vi "Test Properties Report.vi"() -> ()   [LabVIEW 2020]
uses:
  classes/Test Result/Node Results (Extended).ctl
  classes/Test Result/Test Node (Extended).ctl
  classes/Test Result/Test Registration Data.ctl
  classes/Test Result/Assert Event Data (Extended).ctl
  classes/Test Suite/Define Test Suite (JUnit Report).vi
  classes/Test Suite/Define Test Suite (SimpleText Report).vi
  classes/Test Suite/Test Suite.lvclass
  classes/Test Result/Test Result.lvclass
panel:
  out "% Requirement Coverage":dbl
  out "report path":path
  in  "Report Format":enum16{"Basic Text Report", "JUnit Report"}(ring)
  out "Test Results":T1[](array[typedef])
  in  "error in (no error)":errorcluster
  out "error out":errorcluster
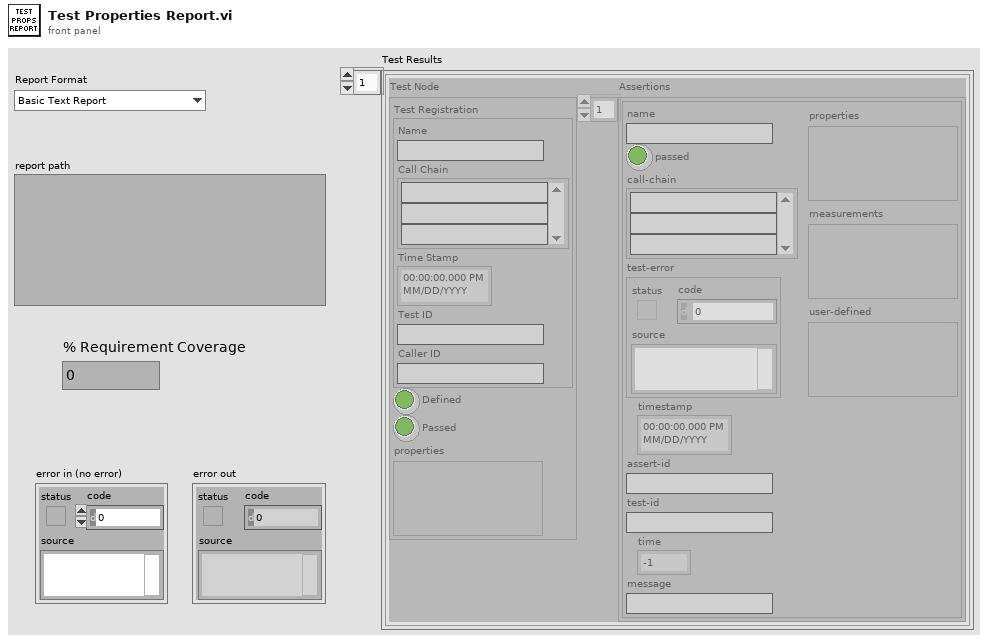
[diagram p1: front panel]
types:
  T1 = typedef "Caraya.lvlib/Test Result.lvclass/Node Results (Extended).ctl" = cluster{"Test Node":T2, "Assertions":T4[]}
  T2 = typedef "Caraya.lvlib/Test Result.lvclass/Test Node (Extended).ctl" = cluster{"Test Registration":T3, "Defined":bool, "Passed":bool, "properties":variant}
  T3 = typedef "Caraya.lvlib/Test Result.lvclass/Test Registration Data.ctl" = cluster{"Name":string, "Call Chain":string[], "Time Stamp":timestamp, "Test ID":string, "Caller ID":string}
  T4 = typedef "Caraya.lvlib/Test Result.lvclass/Assert Event Data (Extended).ctl" = cluster{"name":string, "passed":bool, "call-chain":string[], "test-error":errorcluster, "timestamp":timestamp, "assert-id":string, "test-id":string, "time":dbl, "message":string, "properties":variant, "measurements":variant, "user-defined":variant}
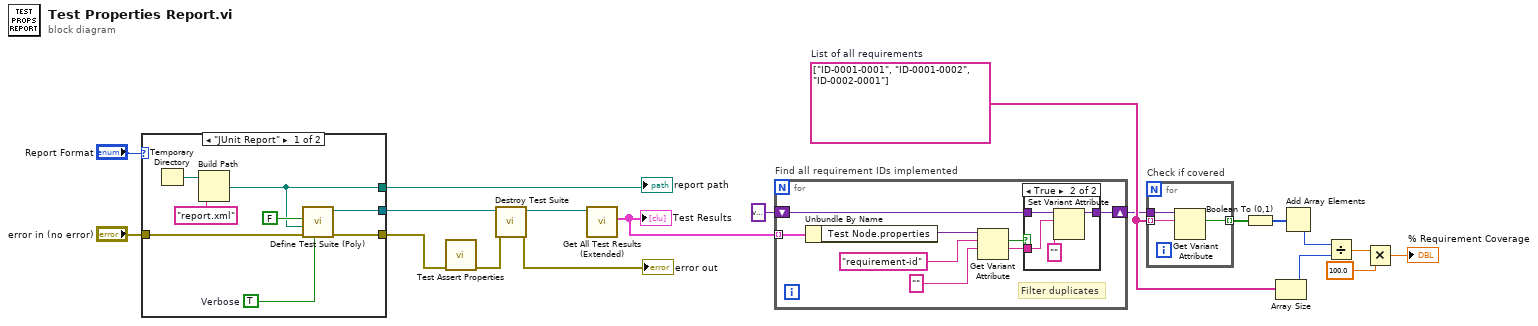
[diagram p0: block diagram]
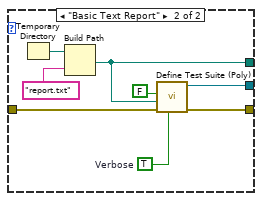
[diagram p3: hidden frame]
diagram:
  w7 = string[] ["ID-0001-0001", "ID-0001-0002", "ID-0002-0001"]  # List of all requirements
  n1 = case shown="\"JUnit Report\"" "Report Format" {
    tunnel: [w25 w35] -> w15
    tunnel: [w22 w32] -> w14
    tunnel: "error in (no error)" -> [w21 w29]
    tunnel: [w20 w28] -> w12
    frame "JUnit Report" {
      w23 = TRUE  # Verbose
      n2 = Temporary Directory() -> (w27:path)
      n3 = Build Path(base path=w27, name or relative path="report.xml") -> (appended path=w22:path)
      n4 = call-poly "Define Test Suite (Poly).vi"("Verbose (F)"=w23, "error in (no error)"=w21, "Report Path"=w22, "Interactive"=FALSE) -> ("error out"=w20:errorcluster, "Test Suite"=w25:refnum<class "Test Suite.lvclass">)  [unwired: 5 in, 1 out]
    }
    frame "Basic Text Report" {
      w31 = TRUE  # Verbose
      n5 = Temporary Directory() -> (w34:path)
      n6 = Build Path(base path=w34, name or relative path="report.txt") -> (appended path=w32:path)
      n7 = call-poly "Define Test Suite (Poly).vi"("Verbose (F)"=w31, "error in (no error)"=w29, "Report Path"=w32, "Interactive"=FALSE) -> ("error out"=w28:errorcluster, "Test Suite"=w35:refnum<class "Test Suite.lvclass">)  [unwired: 5 in, 1 out]
    }
  }
  "report path" <- w14
  n8 = call "Test Assert Properties.vi"("error in (no error)"=w12) -> ("error out"=w17:errorcluster)  [unwired: 10 in]
  n9 = call-dynamic "Destroy Test Suite.vi"("error in (no error)"=w17, "Test Suite in"=w15) -> ("error out"=→"error out":errorcluster, "Test Suite Results"=w19:refnum<class "Test Result.lvclass">)  [unwired: 8 in]
  n10 = call "Get All Test Results (Extended).vi"("Test Result in"=w19) -> ("Test Results"=w11:T1[])  [unwired: 8 in, 2 out]
  "Test Results" <- w11
  n11 = for "Find all requirement IDs implemented" {
    tunnel: w11 -> [w43] mode=indexing
    shift-right: [w38] -> w1
    shift-left: variant -> [w39]
    # "Filter duplicates"
    n12 = Unbundle By Name(w43) -> ("Test Node.properties"=w42:variant)
    n13 = Get Variant Attribute(Variant=w42, name="requirement-id", default value (empty Variant)="") -> (found=w36:bool, value=w37:string)  [unwired: 1 in, 2 out]
    n14 = case shown="True" w36 {
      tunnel: w39 -> [w44 w48]
      tunnel: [w44 w47] -> w38
      tunnel: w37 -> [_ w46]
      frame False {
      }
      frame True {
        n15 = Set Variant Attribute(Variant=w48, name=w46, value="") -> (Variant out=w47:variant)  [unwired: 1 in, 2 out]
      }
    }
  }
  n16 = for "Check if covered" {
    tunnel: w1 -> [w51]
    tunnel: w7 -> [w50] mode=indexing
    tunnel: [w49] -> w9 mode=indexing
    n17 = Get Variant Attribute(Variant=w51, name=w50) -> (found=w49:bool)  [unwired: 2 in, 3 out]
  }
  n18 = Boolean To (0,1)(Boolean=w9) -> (0, 1=w8:i16[])
  n19 = Array Size(array=w7) -> (size(s)=w5:i32)
  n20 = Add Array Elements(numeric array=w8) -> (sum=w6:i16)
  n21 = Divide(x=w6, y=w5) -> (x/y=w4:dbl)
  n22 = Multiply(x=w4, y=100.0) -> (x*y=→"% Requirement Coverage":dbl)
